vi "Long signal copy graph.vi"(8 "エラー入力（エラーなし）":errorcluster, 11 "L Time Profile Table":string[][](table) caption="Time Table") -> (0 "エラー出力":errorcluster, 3 "Time Graph":cluster{"time":dbl[], "current":dbl[]}[](graph))   [LabVIEW 2018]
panel:
  out "Relative Assigned":dbl[](array[numeric])
  out "Relative Raw":dbl[](array[numeric])
  out "Time":dbl[](array[numeric])
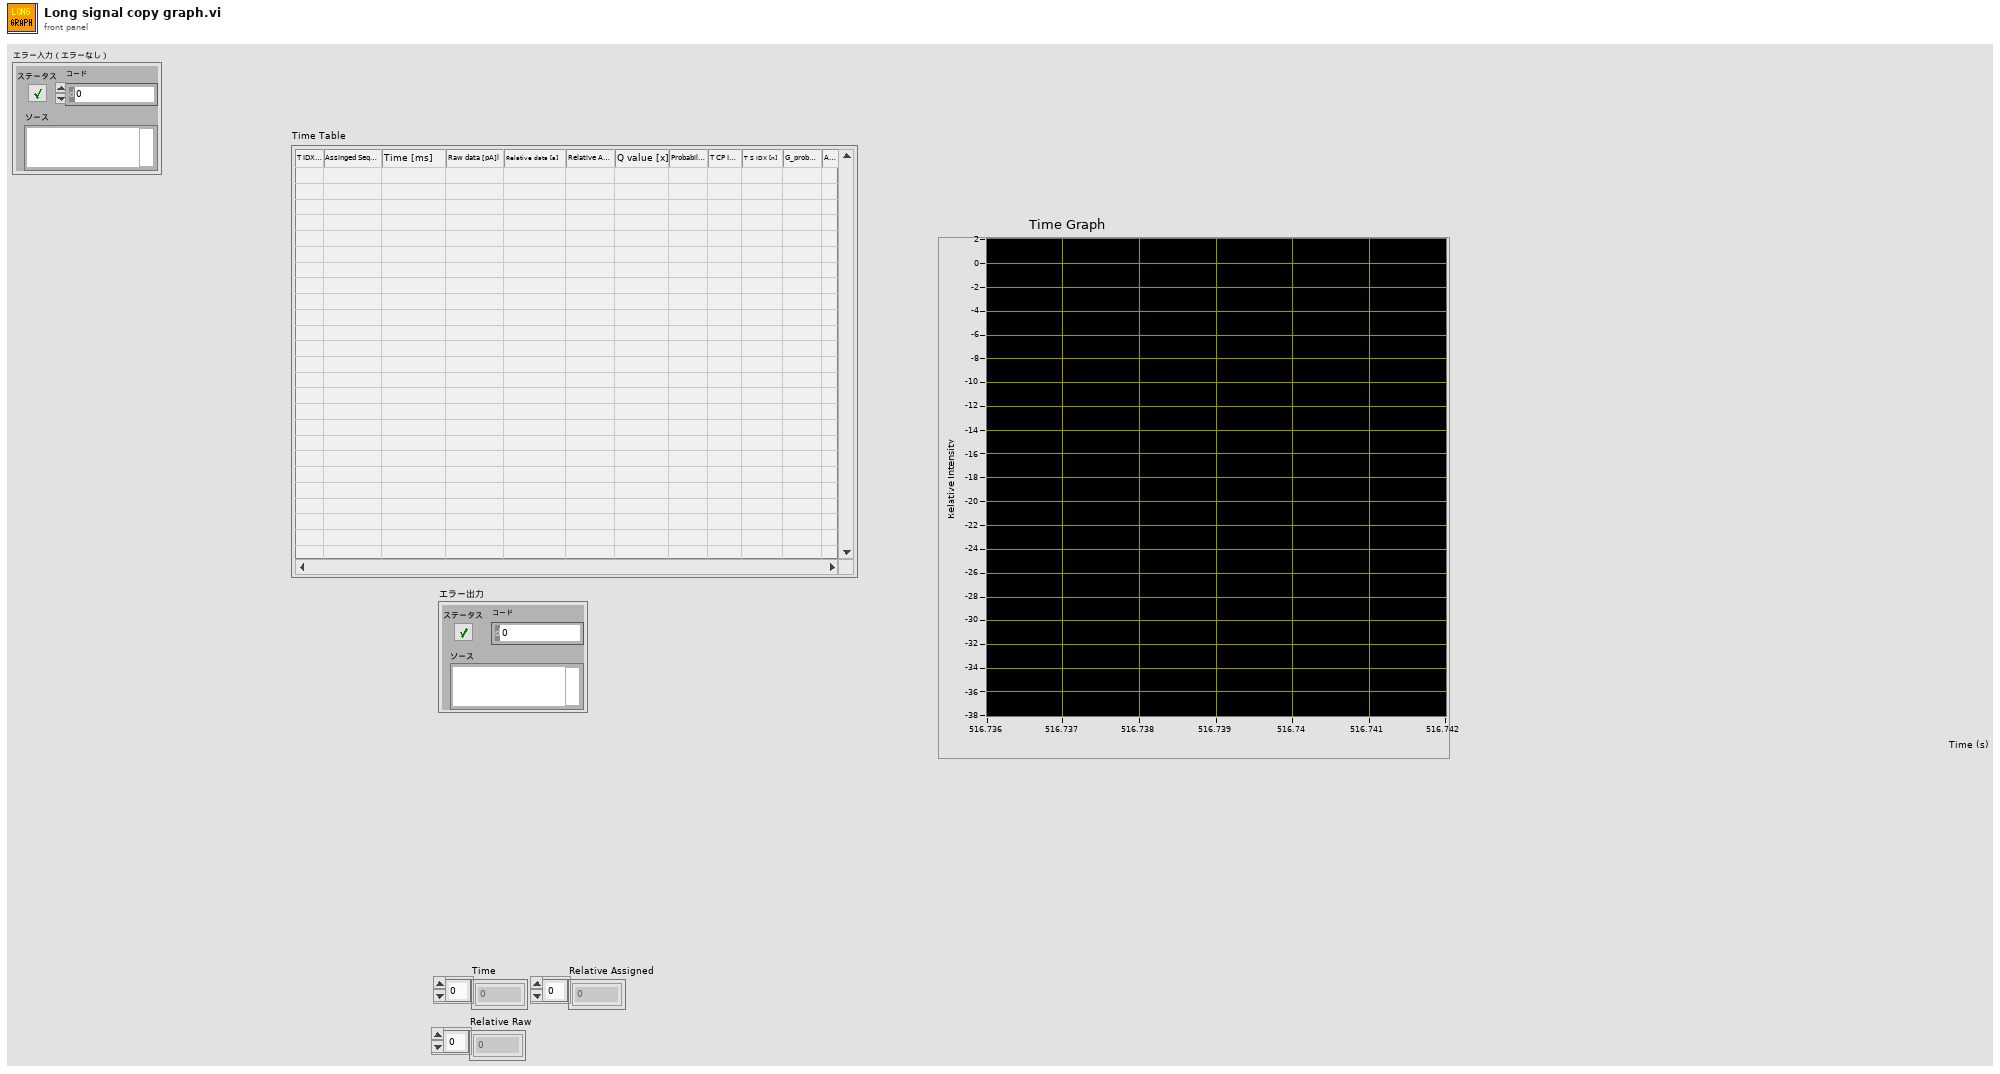
[diagram p1: front panel]
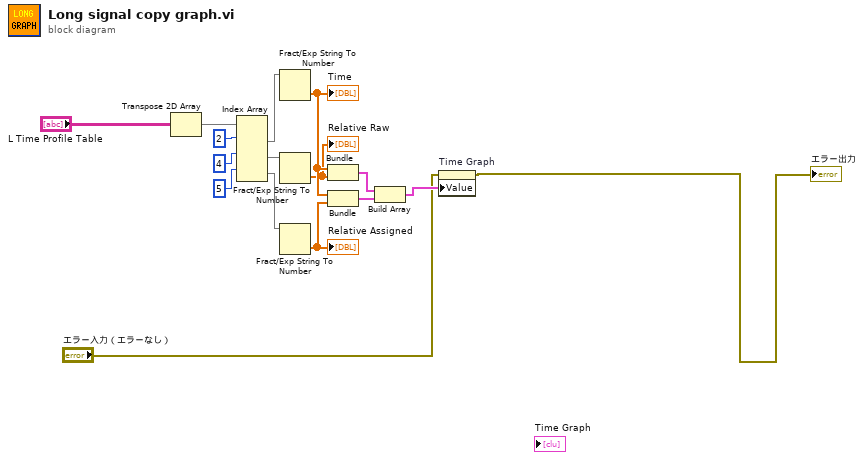
[diagram p0: block diagram]
diagram:
  n1 = Transpose 2D Array(2D array="L Time Profile Table") -> (transposed array=w14:string[][])
  n2 = Index Array(array=w14, index (row) #1=2 ("指標 （行）"), index (row) #2=4 ("指標 （行）"), index (row) #3=5 ("指標 （行）")) -> (element #1=w11:string[], element #2=w9:string[], element #3=w10:string[])  [unwired: 3 in]
  n3 = Fract/Exp String To Number(string=w11) -> (number=w6:dbl[])  [unwired: 3 in, 1 out]
  "Time" <- w6
  n4 = Fract/Exp String To Number(string=w9) -> (number=w5:dbl[])  [unwired: 3 in, 1 out]
  "Relative Raw" <- w5
  n5 = Fract/Exp String To Number(string=w10) -> (number=w4:dbl[])  [unwired: 3 in, 1 out]
  "Relative Assigned" <- w4
  n6 = Bundle(w6, w5) -> (w8:cluster{dbl[], dbl[]})  [unwired: 1 in]
  n7 = Bundle(w6, w4) -> (w7:cluster{dbl[], dbl[]})  [unwired: 1 in]
  n8 = Build Array(w8, w7) -> (w3:cluster{dbl[], dbl[]}[])
  n9 = property on="Time Graph" class="XYGraph (strict)"(error in="エラー入力（エラーなし）", "Value"=w3) -> (error out=→"エラー出力":errorcluster)  [unwired: 1 in, 1 out]
